vi "libssh2_sftp_init.vi"(8 "error in (no error)":errorcluster, 11 "session":T2) -> (0 "error out":errorcluster, 3 "sftp":T1)   [LabVIEW 2017, in "libssh2.lvlib"]
doc: "Initialize an SFTP session."
uses:
  libssh2.lvlib
  Session Refnum.ctl
  SFTP Refnum.ctl
  Not A Session.vi
  <vilib>/Utility/error.llb/Error Cluster From Error Code.vi
  Global Settings.vi
  Read Session Refnum.vi
  <vilib>/Utility/semaphor.llb/Acquire Semaphore.vi
  <vilib>/Utility/semaphor.llb/Release Semaphore.vi
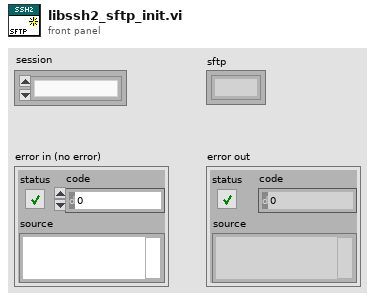
[diagram p1: front panel]
types:
  T1 = typedef "libssh2.lvlib/SFTP Refnum.ctl" = refnum<k1>
  T2 = typedef "libssh2.lvlib/Session Refnum.ctl" = refnum<k1>
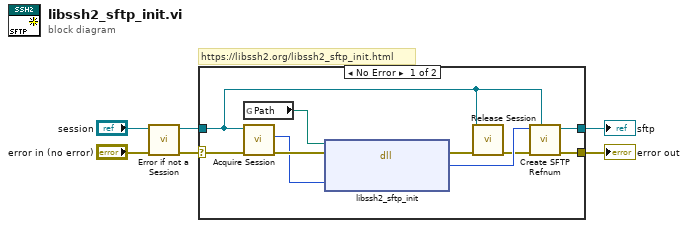
[diagram p0: block diagram]
diagram:
  # "https://libssh2.org/libssh2_sftp_init.html"
  n1 = call "Error if not a Session.vi"("error in (no error)"="error in (no error)", "session"="session") -> ("error out"=w4:errorcluster, "session out"=w3:T2)  [unwired: 8 in]
  n2 = case shown="No Error" w4 {
    selector: w4 -> [w15 w17]
    tunnel: w3 -> [w7 _]
    tunnel: [w11 w17] -> w2
    tunnel: [w9 _] -> w1
    frame No Error {
      n3 = global read "Global Settings.vi" "Path"() -> (w16:path)
      n4 = call "Acquire Session.vi"("error in (no error)"=w15, "session"=w7) -> ("error out"=w14:errorcluster, "LIBSSH2_SESSION*"=w13:u64)  [unwired: 7 in, 1 out]
      n5 = dll-call lib="?" fn="libssh2_sftp_init"(path in=w16, error in=w14, "session"=w13) -> (error out=w12:errorcluster, "return value"=w10:u64)  [unwired: 2 in, 1 out]
      n6 = call "Release Session.vi"("error in (no error)"=w12, "session"=w7) -> ("error out"=w8:errorcluster)  [unwired: 9 in]
      n7 = call "Create SFTP Refnum.vi"("session"=w7, "error in (no error)"=w8, "LIBSSH2_SFTP*"=w10) -> ("error out"=w11:errorcluster, "sftp"=w9:T1)  [unwired: 7 in]
    }
    frame Error {
    }
  }
  "error out" <- w2
  "sftp" <- w1
